vi "RemoteVI Send Static Response.vi"(0 "connection":u32, 5 "status":u16=404, 7 "page?":bool, 9 "html":string) -> (15 "error out":errorcluster)   [LabVIEW 2020, in "RemoteVI.lvlib"]
doc: "Answers an HTTP request that is not a WebSocket upgrade and closes the connection (docs\\protocol.md section 1): status with html as text/html when page? is TRUE, otherwise an empty text/plain body; always with the security headers X-Content-Type-Options, X-Frame-Options, Referrer-Policy, Cache-Control and Content-Security-Policy (docs\\security.md). Built with IG HTTP Utils (Create Basic Response, Set Header, Write Response to TCP). connection is the TCP connection refnum type-cast to U32. Used by RemoteVI Handle Connection.vi."
uses:
  RemoteVI.lvlib
  <vilib>/IlluminatedG/IG HTTP Utils/HTTP Utils/Response/Response.lvclass
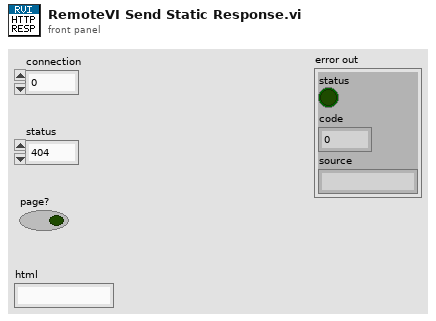
[diagram p1: front panel]
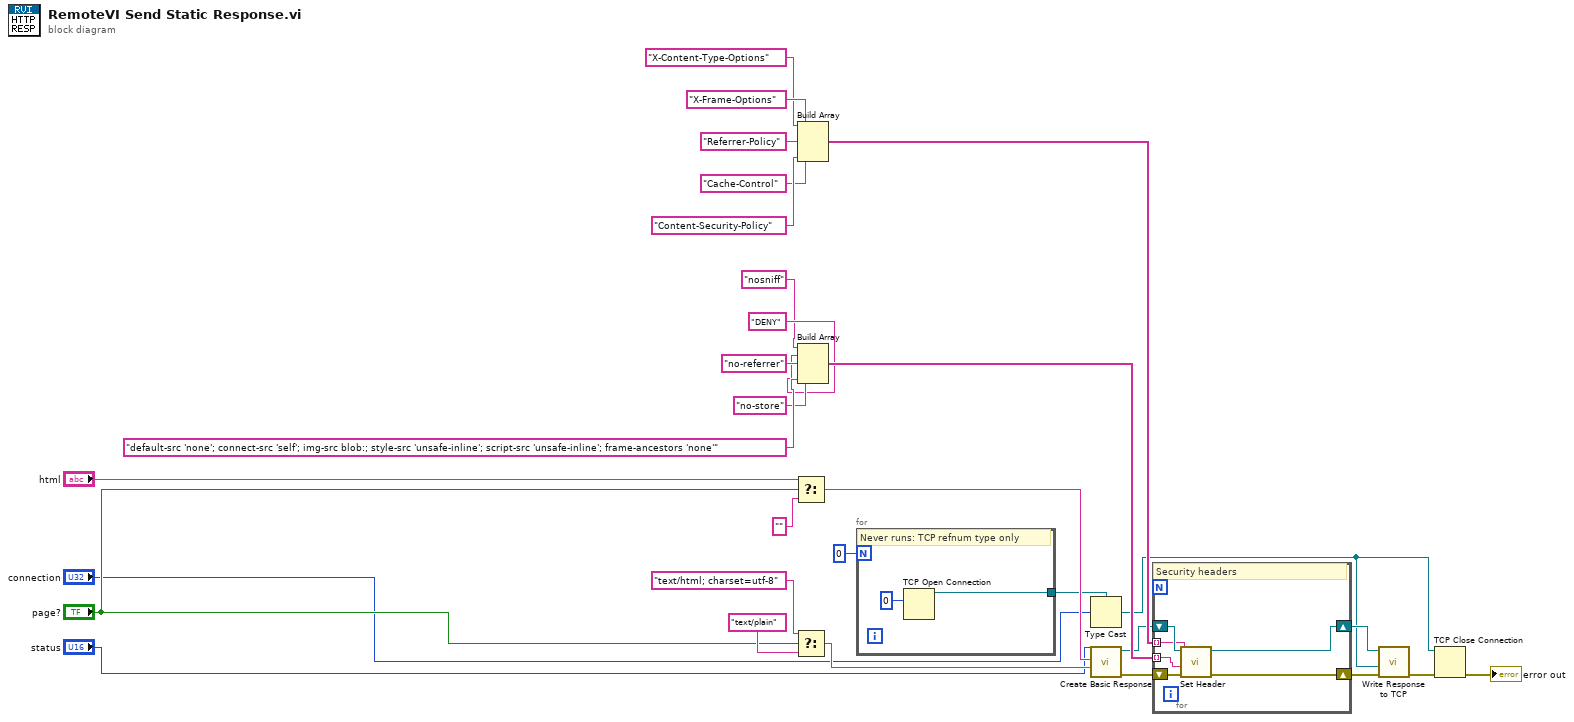
[diagram p0: block diagram]
diagram:
  n1 = Select(t="html", s="page?", f="") -> (s? t:f=w11:string)
  n2 = Select(t="text/html; charset=utf-8", s="page?", f="text/plain") -> (s? t:f=w12:string)
  n3 = Build Array("X-Content-Type-Options", "X-Frame-Options", "Referrer-Policy", "Cache-Control", "Content-Security-Policy") -> (w25:string[])
  n4 = Build Array("nosniff", "DENY", "no-referrer", "no-store", "default-src 'none'; connect-src 'self'; img-src blob:; style-src 'unsafe-inline'; script-src 'unsafe-inline'; frame-ancestors 'none'") -> (w26:string[])
  n5 = for {
    N: 0 -> [_]
    tunnel: [w32] -> w6
    # "Never runs: TCP refnum type only"
    n6 = TCP Open Connection(remote port or service name=u16 0) -> (connection ID=w32:refnum<k5>)  [unwired: 4 in, 1 out]
  }
  n7 = Type Cast(type=w6, x="connection") -> (*(type *) &x=w7:refnum<k5>)
  n8 = call <vilib>:"Create Basic Response.vi"("Content-Type (text/plain)"=w12, "Payload"=w11, "Status Code"="status") -> ("error out"=w13:errorcluster, "Response out"=w14:refnum<class "Response.lvclass">)  [unwired: 7 in]
  n9 = for {
    tunnel: w25 -> [w33] mode=indexing
    tunnel: w26 -> [w34] mode=indexing
    shift-right: [w36] -> w27
    shift-left: w14 -> [w35]
    shift-right: [w38] -> w28
    shift-left: w13 -> [w37]
    # "Security headers"
    n10 = call <vilib>:"Set Header.vi"("error in (no error)"=w37, "Value"=w34, "Header"=w33, "Response in"=w35) -> ("error out"=w38:errorcluster, "Response out"=w36:refnum<class "Response.lvclass">)  [unwired: 5 in, 1 out]
  }
  n11 = call <vilib>:"Write Response to TCP.vi"("error in (no error)"=w28, "TCP Connection"=w7, "Response in"=w27) -> ("error out"=w29:errorcluster)  [unwired: 7 in, 1 out]
  n12 = TCP Close Connection(connection ID=w7, error in (no error)=w29) -> (error out=→"error out":errorcluster)  [unwired: 1 in, 1 out]
